vi "RemoteVI Server.vi"() -> ()   [LabVIEW 2020, in "RemoteVI.lvlib"]
doc: "RemoteVI Server: share any window in a web browser without writing code. Left: the windows that can be shared, LabVIEW's own first, then LabVIEW-built applications, then other programs (LabVIEW windows only narrows the list; it refreshes every 3 s and on Refresh list). Select one, choose the port, Whole network (default: this computer only) and View only, and press Share selected window. Right: the shares of this application instance with their port, reach and clients, live; select one for its details, Stop sharing, Copy link or Open in browser. Every link carries its share's random access token (docs\\security.md). A running VI of this LabVIEW is shared as a VI target, any other window as a window target (RemoteVI Server Share.vi). In LabVIEW (Tools menu) closing the window keeps the shares running; RemoteVI Server.exe stops every share when its window closes, runs a landing page listing the shares (default port 8088, the next free port when that is in use) and reads its command line (RemoteVI Parse Arguments.vi: --share <window title> --port N --token T --whole-network --view-only --landing-port P)."
uses:
  RemoteVI.lvlib
panel:
  in  "Open in browser":bool
  in  "Copy link":bool
  in  "Stop sharing":bool
  in  "View only":bool
  in  "Whole network":bool
  in  "Port":u16=8100
  in  "Share selected window":bool
  in  "LabVIEW windows only":bool
  in  "Refresh list":bool
  in  "tick":bool
  out "Details":string
  out "Message":string
  out "Landing page":string
  in  "Shared now":i32(listbox)
  in  "Windows you can share":i32(listbox)
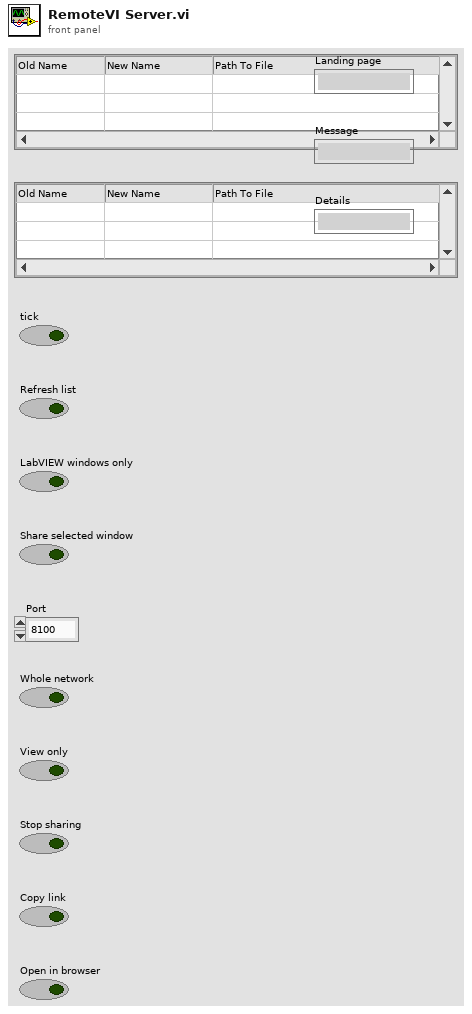
[diagram p1: front panel]
types:
  T1 = cluster{"rows":cluster{"group":i32, "program":string, "title":string, "pid":u32, "hWnd":u64}[], "servers":cluster{"port":u16, "url":string, "target":string, "kind":string, "whole network":bool, "running":bool, "uptime s":dbl, "clients":cluster{"address":string, "connected s":dbl, "idle s":dbl}[], "fps":dbl, "kB per s":dbl, "frames":u32, "latency ms":dbl, "view only":bool, "last error":string, "hWnd":u64}[], "items":string[][], "count":i32, "force":bool, "landing port":u16, "runtime":bool}
  T2 = cluster{"label":string, "left":i32, "top":i32, "width":i32, "height":i32}[]
  T3 = enum32{"invalid app kind", "Development System", "Run Time System", "Student Edition", "Embedded LabVIEW", "Evaluation", "Custom"}
  T4 = cluster{"port":u16, "url":string, "target":string, "kind":string, "whole network":bool, "running":bool, "uptime s":dbl, "clients":cluster{"address":string, "connected s":dbl, "idle s":dbl}[], "fps":dbl, "kB per s":dbl, "frames":u32, "latency ms":dbl, "view only":bool, "last error":string, "hWnd":u64}[]
  T5 = cluster{"share":string, "port":u16, "token":string, "whole network":bool, "view only":bool, "landing port":u16}
  T6 = cluster{"group":i32, "program":string, "title":string, "pid":u32, "hWnd":u64}[]
  T7 = cluster{"group":i32, "program":string, "title":string, "pid":u32, "hWnd":u64}
  T8 = cluster{"port":u16, "url":string, "target":string, "kind":string, "whole network":bool, "running":bool, "uptime s":dbl, "clients":cluster{"address":string, "connected s":dbl, "idle s":dbl}[], "fps":dbl, "kB per s":dbl, "frames":u32, "latency ms":dbl, "view only":bool, "last error":string, "hWnd":u64}
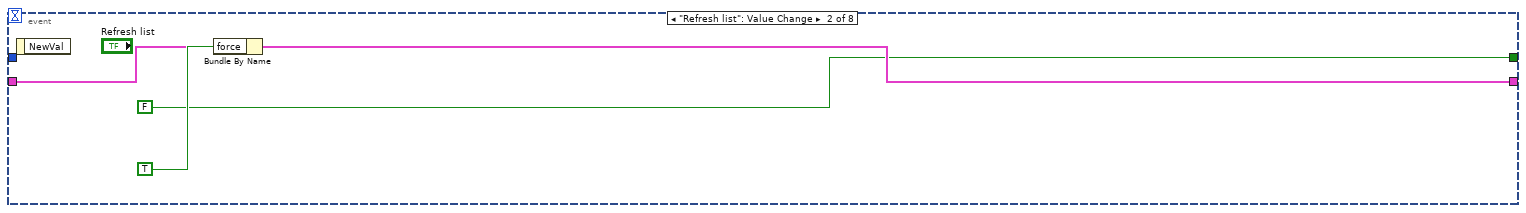
[diagram p4: hidden frame]
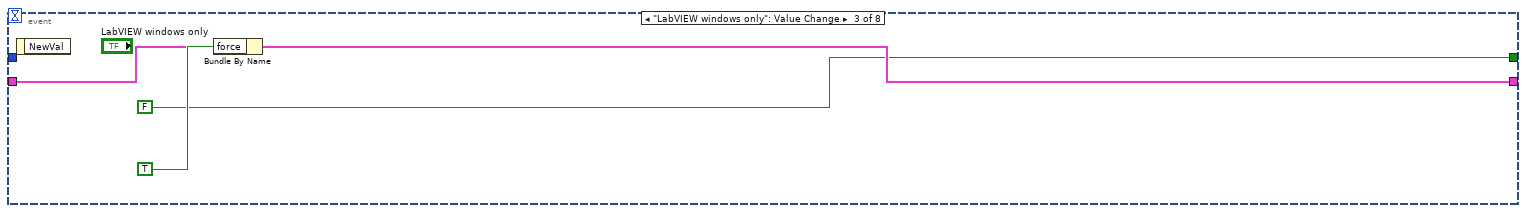
[diagram p5: hidden frame]
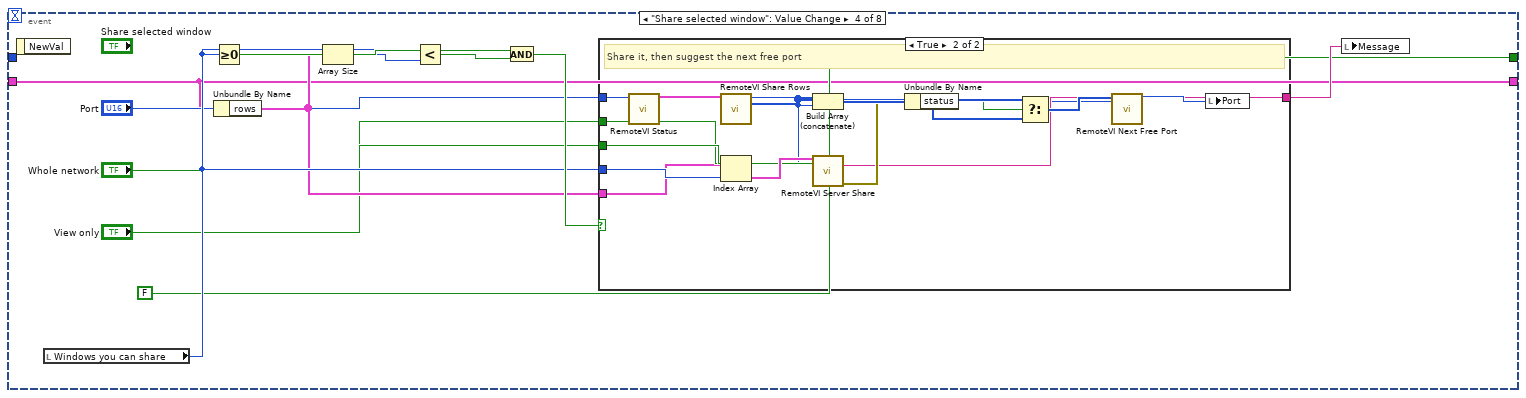
[diagram p6: hidden frame]
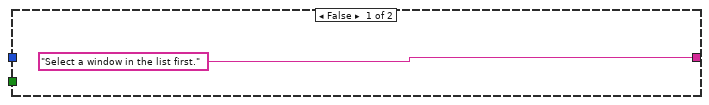
[diagram p7: hidden frame]
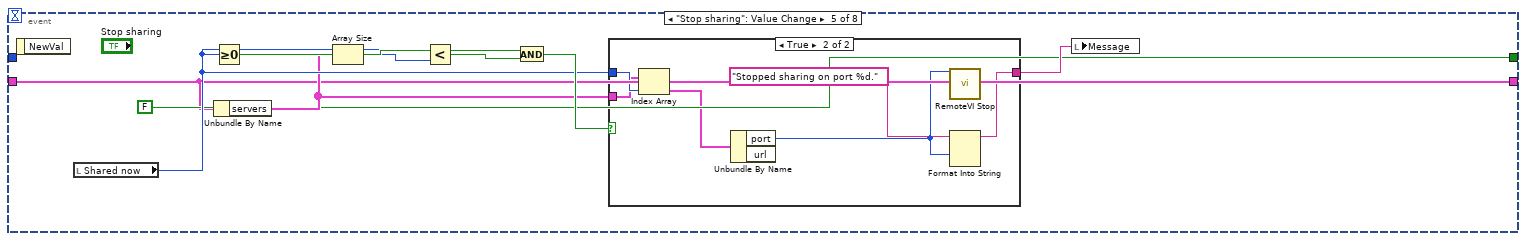
[diagram p8: hidden frame]
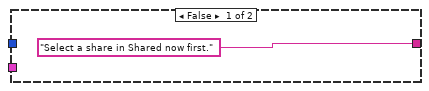
[diagram p9: hidden frame]
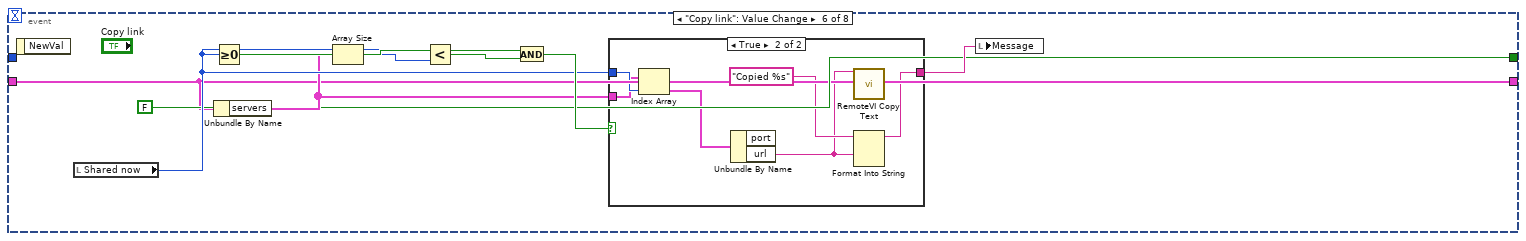
[diagram p10: hidden frame]
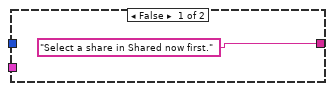
[diagram p11: hidden frame]
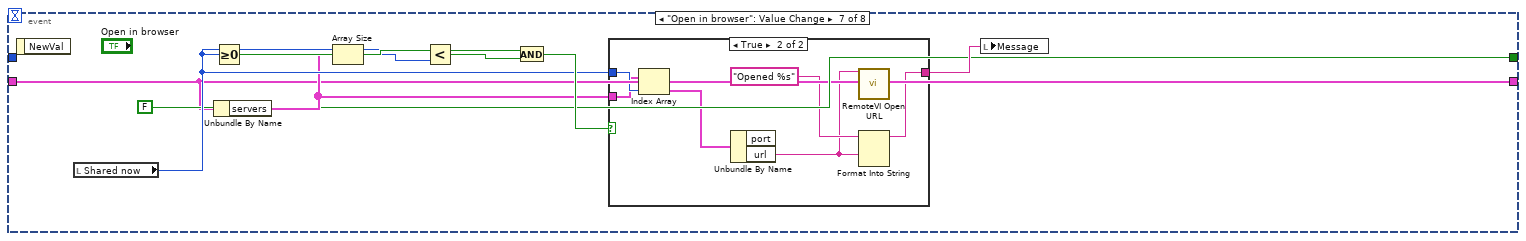
[diagram p12: hidden frame]
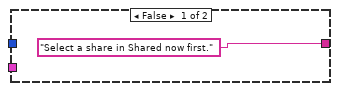
[diagram p13: hidden frame]
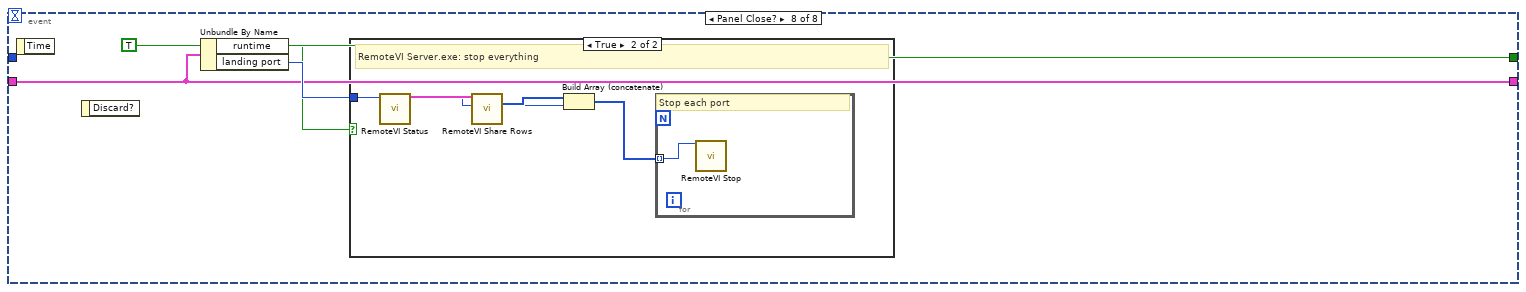
[diagram p14: hidden frame]
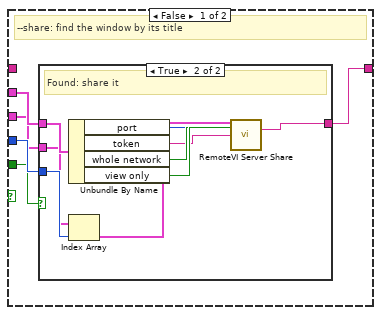
[diagram p17: hidden frame]
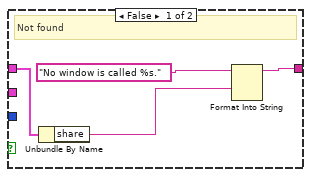
[diagram p18: hidden frame]
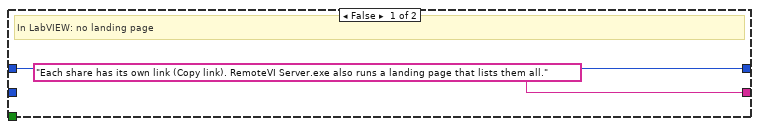
[diagram p19: hidden frame]
diagram:
  w51 = T1 {"rows"=[], "servers"=[], "items"=[], "count"=0, "force"=FALSE, "landing port"=0, "runtime"=FALSE}  # state
  w36 = FALSE
  w31 = u16 0
  w24 = 1
  w22 = 1  # Development System
  w15 = cluster{"list":i32, "column":i32, "width":u32}[] [{"list"=0, "column"=0, "width"=236}, {"list"=0, "column"=1, "width"=120}, {"list"=0, "column"=2, "width"=80}, {"list"=1, "column"=0, "width"=196}, {"list"=1, "column"=1, "width"=46}, {"list"=1, "column"=2, "width"=104}, {"list"=1, "column"=3, "width"=50}]  # column widths
  w9 = TRUE
  w8 = -1
  w4 = "RemoteVI Server"  # title
  w3 = cluster{"width":i32, "height":i32} {"width"=992, "height"=576}  # panel size
  w2 = T2 [{"label"="Windows you can share", "left"=16, "top"=12, "width"=440, "height"=420}, {"label"="LabVIEW windows only", "left"=16, "top"=446, "width"=180, "height"=28}, {"label"="Refresh list", "left"=336, "top"=446, "width"=120, "height"=28}, {"label"="Port", "left"=480, "top"=12, "width"=90, "height"=0}, {"label"="Whole network", "left"=650, "top"=30, "width"=155, "height"=28}, {"label"="View only", "left"=820, "top"=30, "width"=155, "height"=28}, {"label"="Share selected window", "left"=480, "top"=72, "width"=495, "height"=40}, {"label"="Shared now", "left"=480, "top"=126, "width"=440, "height"=170}, {"label"="Stop sharing", "left"=480, "top"=306, "width"=155, "height"=28}, {"label"="Copy link", "left"=650, "top"=306, "width"=155, "height"=28}, {"label"="Open in browser", "left"=820, "top"=306, "width"=155, "height"=28}, {"label"="Details", "left"=480, "top"=346, "width"=495, "height"=128}, {"label"="Message", "left"=16, "top"=488, "width"=960, "height"=24}, {"label"="Landing page", "left"=16, "top"=532, "width"=960, "height"=24}, {"label"="tick", "left"=0, "top"=0, "width"=-1, "height"=0}]  # layout
  # "--share <title>: share that window now"
  n1 = control-ref of="Windows you can share"() -> (w5:refnum<vi>)
  n2 = control-ref of="Shared now"() -> (w13:refnum<vi>)
  n3 = property class="App"() -> ("Application:Kind"=w19:T3, "Application:Command Line Arguments"=w20:string[])  [unwired: 2 in, 2 out]
  n4 = control-ref of="This VI"() -> (w1:refnum<vi>)
  n5 = call "RemoteVI Status.vi"() -> ("servers"=w40:T4)  [unwired: 14 in, 1 out]
  n6 = property class="MCListbox (strict)"(reference=w5, "Number of Columns"=3, "Visible Items:Column Headers Visible"=w9, "Column Header Strings[]"=string[] ["Window", "Program", "Kind"], "Value"=w8) -> (reference out=w12:refnum<vi>)  [unwired: 1 in, 1 out]
  n7 = property class="MCListbox (strict)"(reference=w13, "Number of Columns"=4, "Visible Items:Column Headers Visible"=w9, "Column Header Strings[]"=string[] ["Shared", "Port", "Reach", "Clients"], "Value"=w8) -> (reference out=w14:refnum<vi>)  [unwired: 1 in, 1 out]
  n8 = property class="VI"(reference=w1) -> ("Front Panel Window:OS Window"=w17:i32)  [unwired: 1 in, 2 out]
  n9 = Obtain Notifier(notification data type=FALSE) -> (notifier out=w55:refnum<notifier>)  [unwired: 3 in, 2 out]
  n10 = call "RemoteVI Arrange Controls.vi"("VI"=w1, "layout"=w2, "panel size"=w3, "title"=w4) -> ()  [unwired: 12 in]
  n11 = To Long Integer(number=w19) -> (32bit integer=w21:i32)
  n12 = Array Subset(array=w20, index=w24) -> (w25:string[])  [unwired: 1 in]
  n13 = call "RemoteVI Share Rows.vi"("status"=w40) -> ("ports"=w41:u16[])  [unwired: 13 in, 1 out]
  n14 = while {
    tunnel: w55 -> [w58]
    stop <- w61 stop-if-true
    # "Tick every 500 ms until the event loop ends"
    n15 = Wait on Notification(notifier=w58, timeout in ms (-1)=500) -> (timed out?=w60:bool)  [unwired: 2 in, 3 out]
    n16 = case shown="True" w60 {
      frame False {
      }
      frame True {
        # "Tick: signal the hidden tick control"
        n17 = control-ref of="tick"() -> (w62:refnum<vi>)
        n18 = property class="Bool (strict)"(reference=w62, "Val(Sgnl)"=TRUE) -> ()  [unwired: 1 in, 2 out]
      }
    }
    n19 = Not(x=w60) -> (.not. x?=w61:bool)
  }
  n20 = Build Array(w12, w14) -> (w16:refnum<vi>[])
  n21 = To Unsigned Quad Integer(1:w17) -> (0:w18:u64)
  n22 = Not Equal?(x=w21, y=w22) -> (x != y?=w23:bool)
  n23 = call "RemoteVI Parse Arguments.vi"("args"=w25) -> ("options"=w26:T5)  [unwired: 14 in]
  n24 = for {
    tunnel: w15 -> [w64] mode=indexing
    tunnel: w16 -> [w65]
    # "Column widths"
    n25 = Unbundle By Name(w64) -> ("list"=w66:i32, "column"=w67:i32, "width"=w68:u32)
    n26 = Bundle By Name(cluster=cluster{"Row":i32, "Column":i32} {"Row"=-1, "Column"=0}, "Column"=w67) -> (w71:cluster{"Row":i32, "Column":i32})
    n27 = Index Array(array=w65, index=w66) -> (element=w69:refnum<vi>)
    n28 = property class="MCListbox (strict)"(reference=w69, "Active Cell:Active Cell"=w71, "Cell Size:Width"=w68) -> ()  [unwired: 1 in, 2 out]
  }
  n29 = Unbundle By Name(w26) -> ("share"=w27:string, "port"=w28:u16, "whole network"=w29:bool, "landing port"=w30:u16)  [unwired: 2 out]
  n30 = call "RemoteVI Server Windows.vi"("labview only?"=w36, "skip"=w18, "selected hWnd"=u64 0) -> ("rows"=w38:T6, "items"=w39:string[][])  [unwired: 10 in, 1 out]
  n31 = property class="MCListbox (strict)"(reference=w5, "Item Names"=w39) -> ()  [unwired: 1 in, 2 out]
  n32 = for {
    tunnel: w38 -> [w72] mode=indexing
    tunnel: [w73] -> w43 mode=indexing
    # "Titles"
    n33 = Unbundle By Name(w72) -> ("title"=w73:string)
  }
  n34 = Greater?(x=w30, y=w31) -> (0:w32:bool)
  n35 = call "RemoteVI Next Free Port.vi"("used"=w41, "start"=w28) -> ("port"=w42:u16)  [unwired: 13 in]
  n36 = Empty String/Path?(string/path=w27) -> (empty?=w45:bool)
  n37 = And(x=w23, y=w32) -> (x .and. y?=w33:bool)
  n38 = Search 1D Array(1D array=w43, element=w27) -> (index of element=w44:i32)  [unwired: 1 in]
  n39 = local write "Port"(w42) -> ()
  n40 = case shown="True" w33 {
    tunnel: w31 -> [w74 w78]
    tunnel: w30 -> [_ w76]
    tunnel: w29 -> [_ w77]
    tunnel: [w74 w89] -> w35
    tunnel: ["Each share has its own link (Copy link). RemoteVI Server.exe also runs a landing page that lists them all." w88] -> w34
    frame False {
      # "In LabVIEW: no landing page"
    }
    frame True {
      # "RemoteVI Server.exe: start the landing page"
      n41 = call "RemoteVI Start Landing Page.vi"("whole network?"=w77, "port"=w76) -> ("URL"=w79:string, "port out"=w80:u16, "error out"=w81:errorcluster)  [unwired: 11 in]
      n42 = Unbundle By Name(w81) -> ("status"=w82:bool, "code"=w83:i32)
      n43 = Format Into String(format string="Landing page (a list of every share): %s", w79) -> (resulting string=w85:string)  [unwired: 2 in, 1 out]
      n44 = Format Into String(format string="The landing page did not start (error %d).", w83) -> (resulting string=w87:string)  [unwired: 2 in, 1 out]
      n45 = Select(t=w78, s=w82, f=w80) -> (s? t:f=w89:u16)
      n46 = Select(t=w87, s=w82, f=w85) -> (s? t:f=w88:string)
    }
  }
  "Landing page" <- w34
  n47 = Greater Or Equal?(x=w44, y=0) -> (x >= y?=w47:bool)
  n48 = case shown="True" w45 {
    tunnel: "Select a window, then press Share selected window." -> [_ w108]
    tunnel: [w94 w108] -> w49
    tunnel: w26 -> [w93 _]
    tunnel: w38 -> [w91 _]
    tunnel: w44 -> [w92 _]
    tunnel: w47 -> [w90 _]
    frame False {
      # "--share: find the window by its title"
      n49 = case shown="True" w90 {
        tunnel: w93 -> [w95 w101]
        tunnel: w91 -> [_ w99]
        tunnel: w92 -> [_ w100]
        tunnel: [w98 w107] -> w94
        frame False {
          # "Not found"
          n50 = Unbundle By Name(w95) -> ("share"=w96:string)
          n51 = Format Into String(format string="No window is called %s.", w96) -> (resulting string=w98:string)  [unwired: 2 in, 1 out]
        }
        frame True {
          # "Found: share it"
          n52 = Unbundle By Name(w101) -> ("port"=w103:u16, "token"=w104:string, "whole network"=w105:bool, "view only"=w106:bool)
          n53 = Index Array(array=w99, index=w100) -> (element=w102:T7)
          n54 = call "RemoteVI Server Share.vi"("row"=w102, "port"=w103, "whole network?"=w105, "view only?"=w106, "token"=w104) -> ("message"=w107:string)  [unwired: 8 in, 2 out]
        }
      }
    }
    frame True {
      # "No --share"
    }
  }
  "Message" <- w49
  n55 = Bundle By Name(cluster=w51, "rows"=w38, "servers"=w40, "items"=string[][] [], "count"=w24, "force"=w36, "landing port"=w35, "runtime"=w23) -> (w53:T1)
  n56 = while {
    tunnel: w55 -> [w109]
    tunnel: [w109] -> w56
    tunnel: w18 -> [w110]
    shift-right: [w112] -> _
    shift-left: w53 -> [w111]
    stop <- w113 stop-if-true
    # "Event loop"
    n57 = event shown="[0] \"tick\": Value Change" {
      selector: _ -> [_ _ _ _ _ _ _ _]
      dyn-events: _ -> [_ _ _ _ _ _ _ _]
      timeout: _ -> [_ _ _ _ _ _ _ _]
      tunnel: [FALSE FALSE FALSE FALSE FALSE FALSE FALSE TRUE] -> w113
      tunnel: w110 -> [w115 _ _ _ _ _ _ _]
      tunnel: w111 -> [w114 w157 w161 w165 w192 w208 w224 w240]
      tunnel: [w143 w160 w164 w165 w192 w208 w224 w240] -> w112
      event "tick": Value Change {
        w131 = 1
        n58 = event-data() -> ()  [unwired: 1 in, 1 out]
        n59 = local read "Shared now"() -> (w126:i32)
        n60 = call "RemoteVI Status.vi"() -> ("servers"=w121:T4)  [unwired: 14 in, 1 out]
        n61 = call "RemoteVI Share Rows.vi"("status"=w121) -> ("items"=w122:string[][])  [unwired: 13 in, 1 out]
        n62 = Array Size(array=w121) -> (size(s)=w127:i32)
        n63 = Greater Or Equal To 0?(x=w126) -> (x >= 0?=w128:bool)
        n64 = Array Subset(array=w121, index=w126, length=w131) -> (w132:T4)
        n65 = Unbundle By Name(w114) -> ("rows"=w117:T6, "items"=w118:string[][], "count"=w119:i32, "force"=w120:bool)
        n66 = Flatten To String(anything=w122) -> (data string=w123:string)  [unwired: 3 in, 2 out]
        n67 = Less?(x=w126, y=w127) -> (x < y?=w129:bool)
        n68 = Flatten To String(anything=w118) -> (data string=w124:string)  [unwired: 3 in, 2 out]
        n69 = Quotient & Remainder(x=w119, y=6) -> (x-y*floor(x/y)=w136:i32)  [unwired: 1 out]
        n70 = Add(x=w119, y=w131) -> (x+y=w141:i32)
        n71 = And(x=w128, y=w129) -> (x .and. y?=w130:bool)
        n72 = Not Equal?(x=w123, y=w124) -> (x != y?=w125:bool)
        n73 = Equal?(x=w136, y=0) -> (x = y?=w138:bool)
        n74 = case shown="True" w125 {
          tunnel: w122 -> [_ w155]
          frame False {
          }
          frame True {
            # "Shares changed"
            n75 = control-ref of="Shared now"() -> (w156:refnum<vi>)
            n76 = property class="MCListbox (strict)"(reference=w156, "Item Names"=w155) -> ()  [unwired: 1 in, 2 out]
          }
        }
        n77 = Select(t=w132, s=w130, f=w121) -> (s? t:f=w133:T4)
        n78 = Or(x=w138, y=w120) -> (x .or. y?=w139:bool)
        n79 = case shown="True" w139 {
          tunnel: w115 -> [_ w146]
          tunnel: w117 -> [w144 w145]
          tunnel: [w144 w151] -> w140
          frame False {
          }
          frame True {
            # "Refresh the window list, keep the selected window selected"
            n80 = local read "Windows you can share"() -> (w147:i32)
            n81 = local read "LabVIEW windows only"() -> (w150:bool)
            n82 = control-ref of="Windows you can share"() -> (w154:refnum<vi>)
            n83 = Index Array(array=w145, index=w147) -> (element=w148:T7)
            n84 = Unbundle By Name(w148) -> ("hWnd"=w149:u64)
            n85 = call "RemoteVI Server Windows.vi"("labview only?"=w150, "skip"=w146, "selected hWnd"=w149) -> ("rows"=w151:T6, "items"=w152:string[][], "selected"=w153:i32)  [unwired: 10 in]
            n86 = property class="MCListbox (strict)"(reference=w154, "Item Names"=w152, "Value"=w153) -> ()  [unwired: 1 in, 2 out]
          }
        }
        n87 = call "RemoteVI Status Text.vi"("status"=w133) -> ("text"=w134:string)  [unwired: 14 in]
        n88 = local write "Details"(w134) -> ()
        n89 = Bundle By Name(cluster=w114, "rows"=w140, "servers"=w121, "items"=w122, "count"=w141, "force"=FALSE) -> (w143:T1)
      }
      event "Refresh list": Value Change {
        n90 = event-data() -> ()  [unwired: 1 in, 1 out]
        n91 = Bundle By Name(cluster=w157, "force"=TRUE) -> (w160:T1)
      }
      event "LabVIEW windows only": Value Change {
        n92 = event-data() -> ()  [unwired: 1 in, 1 out]
        n93 = Bundle By Name(cluster=w161, "force"=TRUE) -> (w164:T1)
      }
      event "Share selected window": Value Change {
        n94 = event-data() -> ()  [unwired: 1 in, 1 out]
        n95 = local read "Windows you can share"() -> (w171:i32)
        n96 = Greater Or Equal To 0?(x=w171) -> (x >= 0?=w173:bool)
        n97 = Unbundle By Name(w165) -> ("rows"=w170:T6)
        n98 = Array Size(array=w170) -> (size(s)=w172:i32)
        n99 = Less?(x=w171, y=w172) -> (x < y?=w174:bool)
        n100 = And(x=w173, y=w174) -> (x .and. y?=w175:bool)
        n101 = case shown="True" w175 {
          tunnel: "Port" -> [_ w180]
          tunnel: "Whole network" -> [_ w181]
          tunnel: "View only" -> [_ w182]
          tunnel: w171 -> [_ w179]
          tunnel: w170 -> [_ w178]
          tunnel: ["Select a window in the list first." w184] -> w176
          frame False {
          }
          frame True {
            # "Share it, then suggest the next free port"
            n102 = call "RemoteVI Status.vi"() -> ("servers"=w187:T4)  [unwired: 14 in, 1 out]
            n103 = call "RemoteVI Share Rows.vi"("status"=w187) -> ("ports"=w188:u16[])  [unwired: 13 in, 1 out]
            n104 = Index Array(array=w178, index=w179) -> (element=w183:T7)
            n105 = Build Array (concatenate)(w188, w180) -> (w189:u16[])
            n106 = call "RemoteVI Server Share.vi"("row"=w183, "port"=w180, "whole network?"=w181, "view only?"=w182) -> ("message"=w184:string, "error out"=w185:errorcluster)  [unwired: 9 in, 1 out]
            n107 = Unbundle By Name(w185) -> ("status"=w186:bool)
            n108 = Select(t=w188, s=w186, f=w189) -> (s? t:f=w190:u16[])
            n109 = call "RemoteVI Next Free Port.vi"("used"=w190, "start"=w180) -> ("port"=w191:u16)  [unwired: 13 in]
            n110 = local write "Port"(w191) -> ()
          }
        }
        n111 = local write "Message"(w176) -> ()
      }
      event "Stop sharing": Value Change {
        n112 = event-data() -> ()  [unwired: 1 in, 1 out]
        n113 = local read "Shared now"() -> (w195:i32)
        n114 = Greater Or Equal To 0?(x=w195) -> (x >= 0?=w197:bool)
        n115 = Unbundle By Name(w192) -> ("servers"=w194:T4)
        n116 = Array Size(array=w194) -> (size(s)=w196:i32)
        n117 = Less?(x=w195, y=w196) -> (x < y?=w198:bool)
        n118 = And(x=w197, y=w198) -> (x .and. y?=w199:bool)
        n119 = case shown="True" w199 {
          tunnel: w195 -> [_ w203]
          tunnel: w194 -> [_ w202]
          tunnel: ["Select a share in Shared now first." w207] -> w200
          frame False {
          }
          frame True {
            n120 = Index Array(array=w202, index=w203) -> (element=w204:T8)
            n121 = Unbundle By Name(w204) -> ("port"=w205:u16)  [unwired: 1 out]
            n122 = call "RemoteVI Stop.vi"("port"=w205) -> ()  [unwired: 14 in, 1 out]
            n123 = Format Into String(format string="Stopped sharing on port %d.", w205) -> (resulting string=w207:string)  [unwired: 2 in, 1 out]
          }
        }
        n124 = local write "Message"(w200) -> ()
      }
      event "Copy link": Value Change {
        n125 = event-data() -> ()  [unwired: 1 in, 1 out]
        n126 = local read "Shared now"() -> (w211:i32)
        n127 = Greater Or Equal To 0?(x=w211) -> (x >= 0?=w213:bool)
        n128 = Unbundle By Name(w208) -> ("servers"=w210:T4)
        n129 = Array Size(array=w210) -> (size(s)=w212:i32)
        n130 = Less?(x=w211, y=w212) -> (x < y?=w214:bool)
        n131 = And(x=w213, y=w214) -> (x .and. y?=w215:bool)
        n132 = case shown="True" w215 {
          tunnel: w211 -> [_ w219]
          tunnel: w210 -> [_ w218]
          tunnel: ["Select a share in Shared now first." w223] -> w216
          frame False {
          }
          frame True {
            n133 = Index Array(array=w218, index=w219) -> (element=w220:T8)
            n134 = Unbundle By Name(w220) -> ("url"=w221:string)  [unwired: 1 out]
            n135 = call "RemoteVI Copy Text.vi"("text"=w221) -> ()  [unwired: 14 in, 1 out]
            n136 = Format Into String(format string="Copied %s", w221) -> (resulting string=w223:string)  [unwired: 2 in, 1 out]
          }
        }
        n137 = local write "Message"(w216) -> ()
      }
      event "Open in browser": Value Change {
        n138 = event-data() -> ()  [unwired: 1 in, 1 out]
        n139 = local read "Shared now"() -> (w227:i32)
        n140 = Greater Or Equal To 0?(x=w227) -> (x >= 0?=w229:bool)
        n141 = Unbundle By Name(w224) -> ("servers"=w226:T4)
        n142 = Array Size(array=w226) -> (size(s)=w228:i32)
        n143 = Less?(x=w227, y=w228) -> (x < y?=w230:bool)
        n144 = And(x=w229, y=w230) -> (x .and. y?=w231:bool)
        n145 = case shown="True" w231 {
          tunnel: w227 -> [_ w235]
          tunnel: w226 -> [_ w234]
          tunnel: ["Select a share in Shared now first." w239] -> w232
          frame False {
          }
          frame True {
            n146 = Index Array(array=w234, index=w235) -> (element=w236:T8)
            n147 = Unbundle By Name(w236) -> ("url"=w237:string)  [unwired: 1 out]
            n148 = call "RemoteVI Open URL.vi"("URL"=w237) -> ()  [unwired: 14 in, 1 out]
            n149 = Format Into String(format string="Opened %s", w237) -> (resulting string=w239:string)  [unwired: 2 in, 1 out]
          }
        }
        n150 = local write "Message"(w232) -> ()
      }
      event Panel Close? {
        n151 = event-data() -> ()  [unwired: 1 in, 1 out]
        n152 = event-data() -> ()  [unwired: 2 in, 1 out]
        n153 = Unbundle By Name(w240) -> ("runtime"=w241:bool, "landing port"=w242:u16)
        n154 = case shown="True" w241 {
          tunnel: w242 -> [_ w244]
          frame False {
            # "In LabVIEW the shares keep running"
          }
          frame True {
            # "RemoteVI Server.exe: stop everything"
            n155 = call "RemoteVI Status.vi"() -> ("servers"=w245:T4)  [unwired: 14 in, 1 out]
            n156 = call "RemoteVI Share Rows.vi"("status"=w245) -> ("ports"=w246:u16[])  [unwired: 13 in, 1 out]
            n157 = Build Array (concatenate)(w246, w244) -> (w247:u16[])
            n158 = for {
              tunnel: w247 -> [w248] mode=indexing
              # "Stop each port"
              n159 = call "RemoteVI Stop.vi"("port"=w248) -> ()  [unwired: 14 in, 1 out]
            }
          }
        }
      }
    }
  }
  n160 = Send Notification(notification=w9, notifier=w56) -> (notifier out=w57:refnum<notifier>)  [unwired: 1 in, 1 out]
  n161 = Release Notifier(notifier=w57) -> ()  [unwired: 2 in, 3 out]
  "Details" <- ""
